vi "CSM - Remove all CSM Bookmarks.vi"   [LabVIEW 2017]
doc: "Remove all bookmarks in the CSM module."
uses:
  _ui/csm-ui-support.lvlib
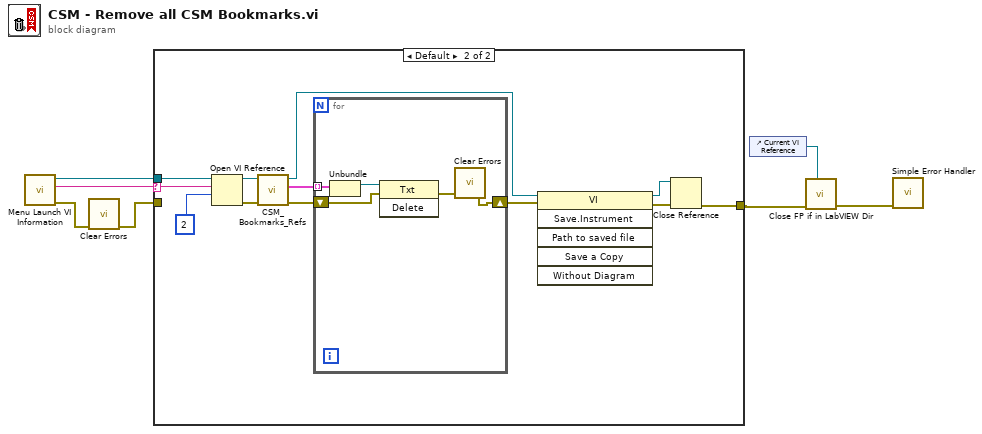
[diagram p0: block diagram]
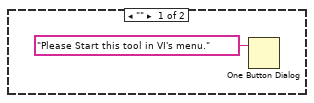
[diagram p2: hidden frame]
diagram:
  n1 = call <vilib>:"Menu Launch VI Information.vi"() -> ("error out"=w5:errorcluster, "Menu Launch:VI"=w6:string, "Menu Launch:App"=w7:refnum<vi>)  [unwired: 9 in]
  n2 = call <vilib>:"Clear Errors.vi"("error in (no error)"=w5) -> ("error out"=w4:errorcluster)  [unwired: 5 in, 1 out]
  n3 = case shown="Default" w6 {
    selector: w6 -> [_ w14]
    tunnel: w7 -> [_ w15]
    tunnel: [_ w9] -> w2
    tunnel: w4 -> [_ _]
    frame "" {
      n4 = One Button Dialog(message="Please Start this tool in VI's menu.") -> ()  [unwired: 1 in, 1 out]
    }
    frame Default {
      n5 = Open VI Reference(application reference (local)=w15, vi path=w14, options=2) -> (vi reference=w20:refnum<vi>, error out=w12:errorcluster)  [unwired: 3 in]
      n6 = call "CSM_Bookmarks_Refs.vi"("error in (no error)"=w12, "VIRef"=w20) -> ("error out"=w18:errorcluster, "Array"=w19:cluster{refnum<vi>, "Text":string}[], "Reference Out"=w16:refnum<vi>)  [unwired: 7 in]
      n7 = for {
        tunnel: w19 -> [w25] mode=indexing
        shift-right: [w21] -> w17
        shift-left: w18 -> [w23]
        n8 = Unbundle(w25) -> (w24:refnum<vi>)  [unwired: 1 out]
        n9 = invoke class="Txt" method="Delete"(reference=w24, error in=w23) -> (error out=w22:errorcluster)  [unwired: 1 in, 2 out]
        n10 = call <vilib>:"Clear Errors.vi"("error in (no error)"=w22) -> ("error out"=w21:errorcluster)  [unwired: 5 in, 1 out]
      }
      n11 = invoke class="VI" method="Save.Instrument"(reference=w16, error in=w17) -> (reference out=w11:refnum<vi>, error out=w10:errorcluster)  [unwired: 4 in, 4 out]
      n12 = Close Reference(reference=w11, error in (no error)=w10) -> (error out=w9:errorcluster)
    }
  }
  n13 = control-ref of="Current VI Reference"() -> (w3:refnum<vi>)
  n14 = call "Close FP if in LabVIEW Dir.vi"("VI Refnum"=w3, "Error in"=w2) -> ("Error out"=w1:errorcluster)  [unwired: 9 in]
  n15 = call <vilib>:"Simple Error Handler.vi"("error in (no error)"=w1) -> ()  [unwired: 4 in, 5 out]
